vi "20180816 1st Step Analysis.vi"(8 "error in":errorcluster caption="エラー入力", 10 "Set Condition":T8={"+/- Point"=2000, "Cut Region"=500, "BL Selection"=enum."Div Value Mode BL", "STD Selection"=enum."DivSTD Mode STD", "D Th std xn"=1.0, "U Th std xn"=6.0, "MAX D time (ms)"=10.0, "LL BR (n)"=0, "LL BR T length (ms)"=0.0, "LL Retention (ms)"=0.0, "Read Region Point"=10000, "Filter Selection"=enum."Smooth", "STD smooth Point"=10, "MAX E_S time (ms)"=10.0}, 11 "F_name":path=path "D:/MCBJ data/Micro RNA Data/let7f W22/00 Good Signal") -> (0 "error out":errorcluster caption="エラー出力", 2 "Count Graph":cluster{i32[], "Count":dbl[]}[](graph), 3 "Raw data Graph":waveform(dbl)(graph))   [LabVIEW 2018]
uses:
  <vilib>/Analysis/NI_AALBase.lvlib
panel:
  out "stripped path":path
  out "path 2":path
  out "path":path
  out "A New Folder temp":string
  out "Table tmp cluster":T1
  out "Path_Name":T2
  out "tdms tmp path":path
  out "R Pre Burst#":i32
  out "S Table Z":T3
  out "S Anal":cluster{string[], string[], string[]}
  out "Total Burst (s)":dbl
  out "Burst S (n)":i32
  out "AR Table Data":string[](array[string])
  out "AR Table Tag":string[](array[string])
  out "Table Pass refnum":T4
  out "Table Tag C":T5
  out "AA2 info":T6
  out "AR Table Path":path
  out "AA info":T7
  out "before":string
  out "1s datapoint":i32
  in  "Selection":enum16{"10kHz", "100kHz"}(ring)
  out "AC Table Data":string[](array[string])
  out "AC Table Tag":string[](array[string])
  in  "Cut Region":i32=500
  out "info Cluster":T9
  out "R B_SCount [n] in":i32
  out "B Region Time [s] in":dbl
  out "JPEG Path":path
  in  "Region Count":dbl[](array[numeric])
  out "Region BL":dbl[](array[numeric])
  out "TDMS temp refnum":refnum<k34>
  out "S_save C":T10
  out "R Table refnum":refnum<file>
  out "B Table refnum":refnum<file>
  out "S Table refnum":refnum<file>
  out "Burst Pre Count":i32
  out "S Peak Position Final (s)":dbl=1000.0 format="%#_13g"
  out "Signal Pre Count":i32
  out "A TDMS Path":path
  out "B Table Path":path
  out "D con":string
  out "A New folder":string
  out "B Table Tag":string[](array[string])
  out "R Table Tag":string[](array[string])
  out "S Table Tag":string[](array[string])
  out "Burst Array":T11
  out "Burst#Sum":i32
  out "BCC":T12
  in  "MAX E_S time(s)":dbl=0.01 format="%#_13g"
  out "BL and Raw":T13
  in  "LL BR (n)":i32
  in  "LL BR T length (ms)":dbl
  out "Under D array":T14
  out "Peak#":i32
  in  "MAX D time(s)":dbl=0.01 format="%#_13g"
  out "Peak Array":T15
  in  "control":enum32{"Signal", "Region"}(tab)
  out "STD Graph":cluster{i32[], "Count":dbl[]}[](graph)
  out "BL Graph":cluster{i32[], "Count":dbl[]}[](graph)
  out "A Cluster":T16
  out "Signal Freq [/s]":dbl format="%#_4g"
  out "Anal Time":string
  out "Signal TT Graph":T17(graph)
  out "Histogram Graph":T18(graph) caption="ヒストグラムグラフ"
  out "Signal-Time Plot":T19(graph)
  out "Signal-Duration Plot":cluster{i32[], dbl[]}(graph)
  out "Burst Time Profile":cluster{i32[], "SDS":dbl[]}[](graph)
  out "Region Info":T20
  out "AN time":string
  out "Ainfo":string
  out "F ex Info":T21
  out "Ex Time":i32
  out "R Table Path":path
  out "S Table Path":path
  in  "LL Retention (ms)":dbl
  in  "Analysis Table TAB":T22(tab)
  out "S Table":string[][](table)
  out "R Table":string[][](table)
  out "B Table":string[][](table)
  in  "Filter Selection":enum16{"Mean", "Smooth"}(ring)=enum."Smooth"
  in  "+/- Point":i32=2000
  out "Region Raw data":dbl[](array[numeric])
  out "Estimated BL":dbl[](array[numeric])
  out "Substracted Raw data":dbl[](array[numeric])
  in  "BL Selection":T23(ring)=enum."Div Value Mode BL"
  out "Selected Region BL":dbl
  in  "STD Selection":T24(ring)=enum."DivSTD Mode STD"
  out "Selected STD (pA)":dbl
  in  "U Th std xn":dbl=6.0 format="%#_13g"
  in  "D Th std xn":dbl=1.0 format="%#_13g"
  out "Region graph":cluster{"Value":i32[], "UP Thre Func":dbl[]}[](graph)
  out "R Peak location":i32[](array[numeric])
  out "Peak Y":dbl[](array[numeric])
  out "U thred (pA)":dbl
  out "D thred (pA)":dbl
  out "UP Thre Func":dbl[](array[numeric])
  out "Peak G":cluster{"Value":i32[], "Peak Y":dbl[]}
  out "Time for Graph":i32[](array[numeric])
  out "Threshold G":cluster{"Value":i32[], "UP Thre Func":dbl[]}
  out "Raw G":cluster{"Value":i32[], "Peak Y":dbl[]}
  out "BL G":cluster{"Value":i32[], "Value":dbl[]}
  out "Peak Intensity":dbl[](array[numeric])
  out "RS Start":i32[](array[numeric])
  out "RS End":i32[](array[numeric])
  out "Signal Time (ms)":dbl[](array[numeric])
  out "Region Start":i32
  out "TS Peak Time (s)":dbl[](array[numeric])
  out "T Start Time (s)":dbl[](array[numeric])
  out "T END Time (s)":dbl[](array[numeric])
  out "Signal location BL":dbl[](array[numeric])
  out "Filter Select":string
  out "Region BL select":string
  out "R STD select":string
  out "S Table C2":T25={"R BL (pA)"=0.0, "R STD (pA)"=0.0, "U thre (pA)"=0.0, "D thre (pA)"=0.0, "U thre (n)"=0.0, "D thre (n)"=0.0, "STD smoth Point "=10, "MAX Duration time(s)"=0.01} {"MAX Duration time(s)" format="%#_13g"}
  out "S Table C1":T26
  out "S Table C0":T27
  out "Rigon#":i32
  out "BL cluster":T28
  out "HPeak Cluster":T29
  out "STD cluster":T30
  out "R Table C0":T31
  in  "STD smooth Point":i32=10
  out "Signal#Sum":i32
  out "Raw data":dbl[](array[numeric])
  out "Filename":string
  in  "Read Region Point":i32=10000
  out "datapoint":i32
  out "Region STD":dbl[](array[numeric])
  out "Count":dbl[](array[numeric])
  out "STD":dbl[](array[numeric])
  out "BL":dbl[](array[numeric])
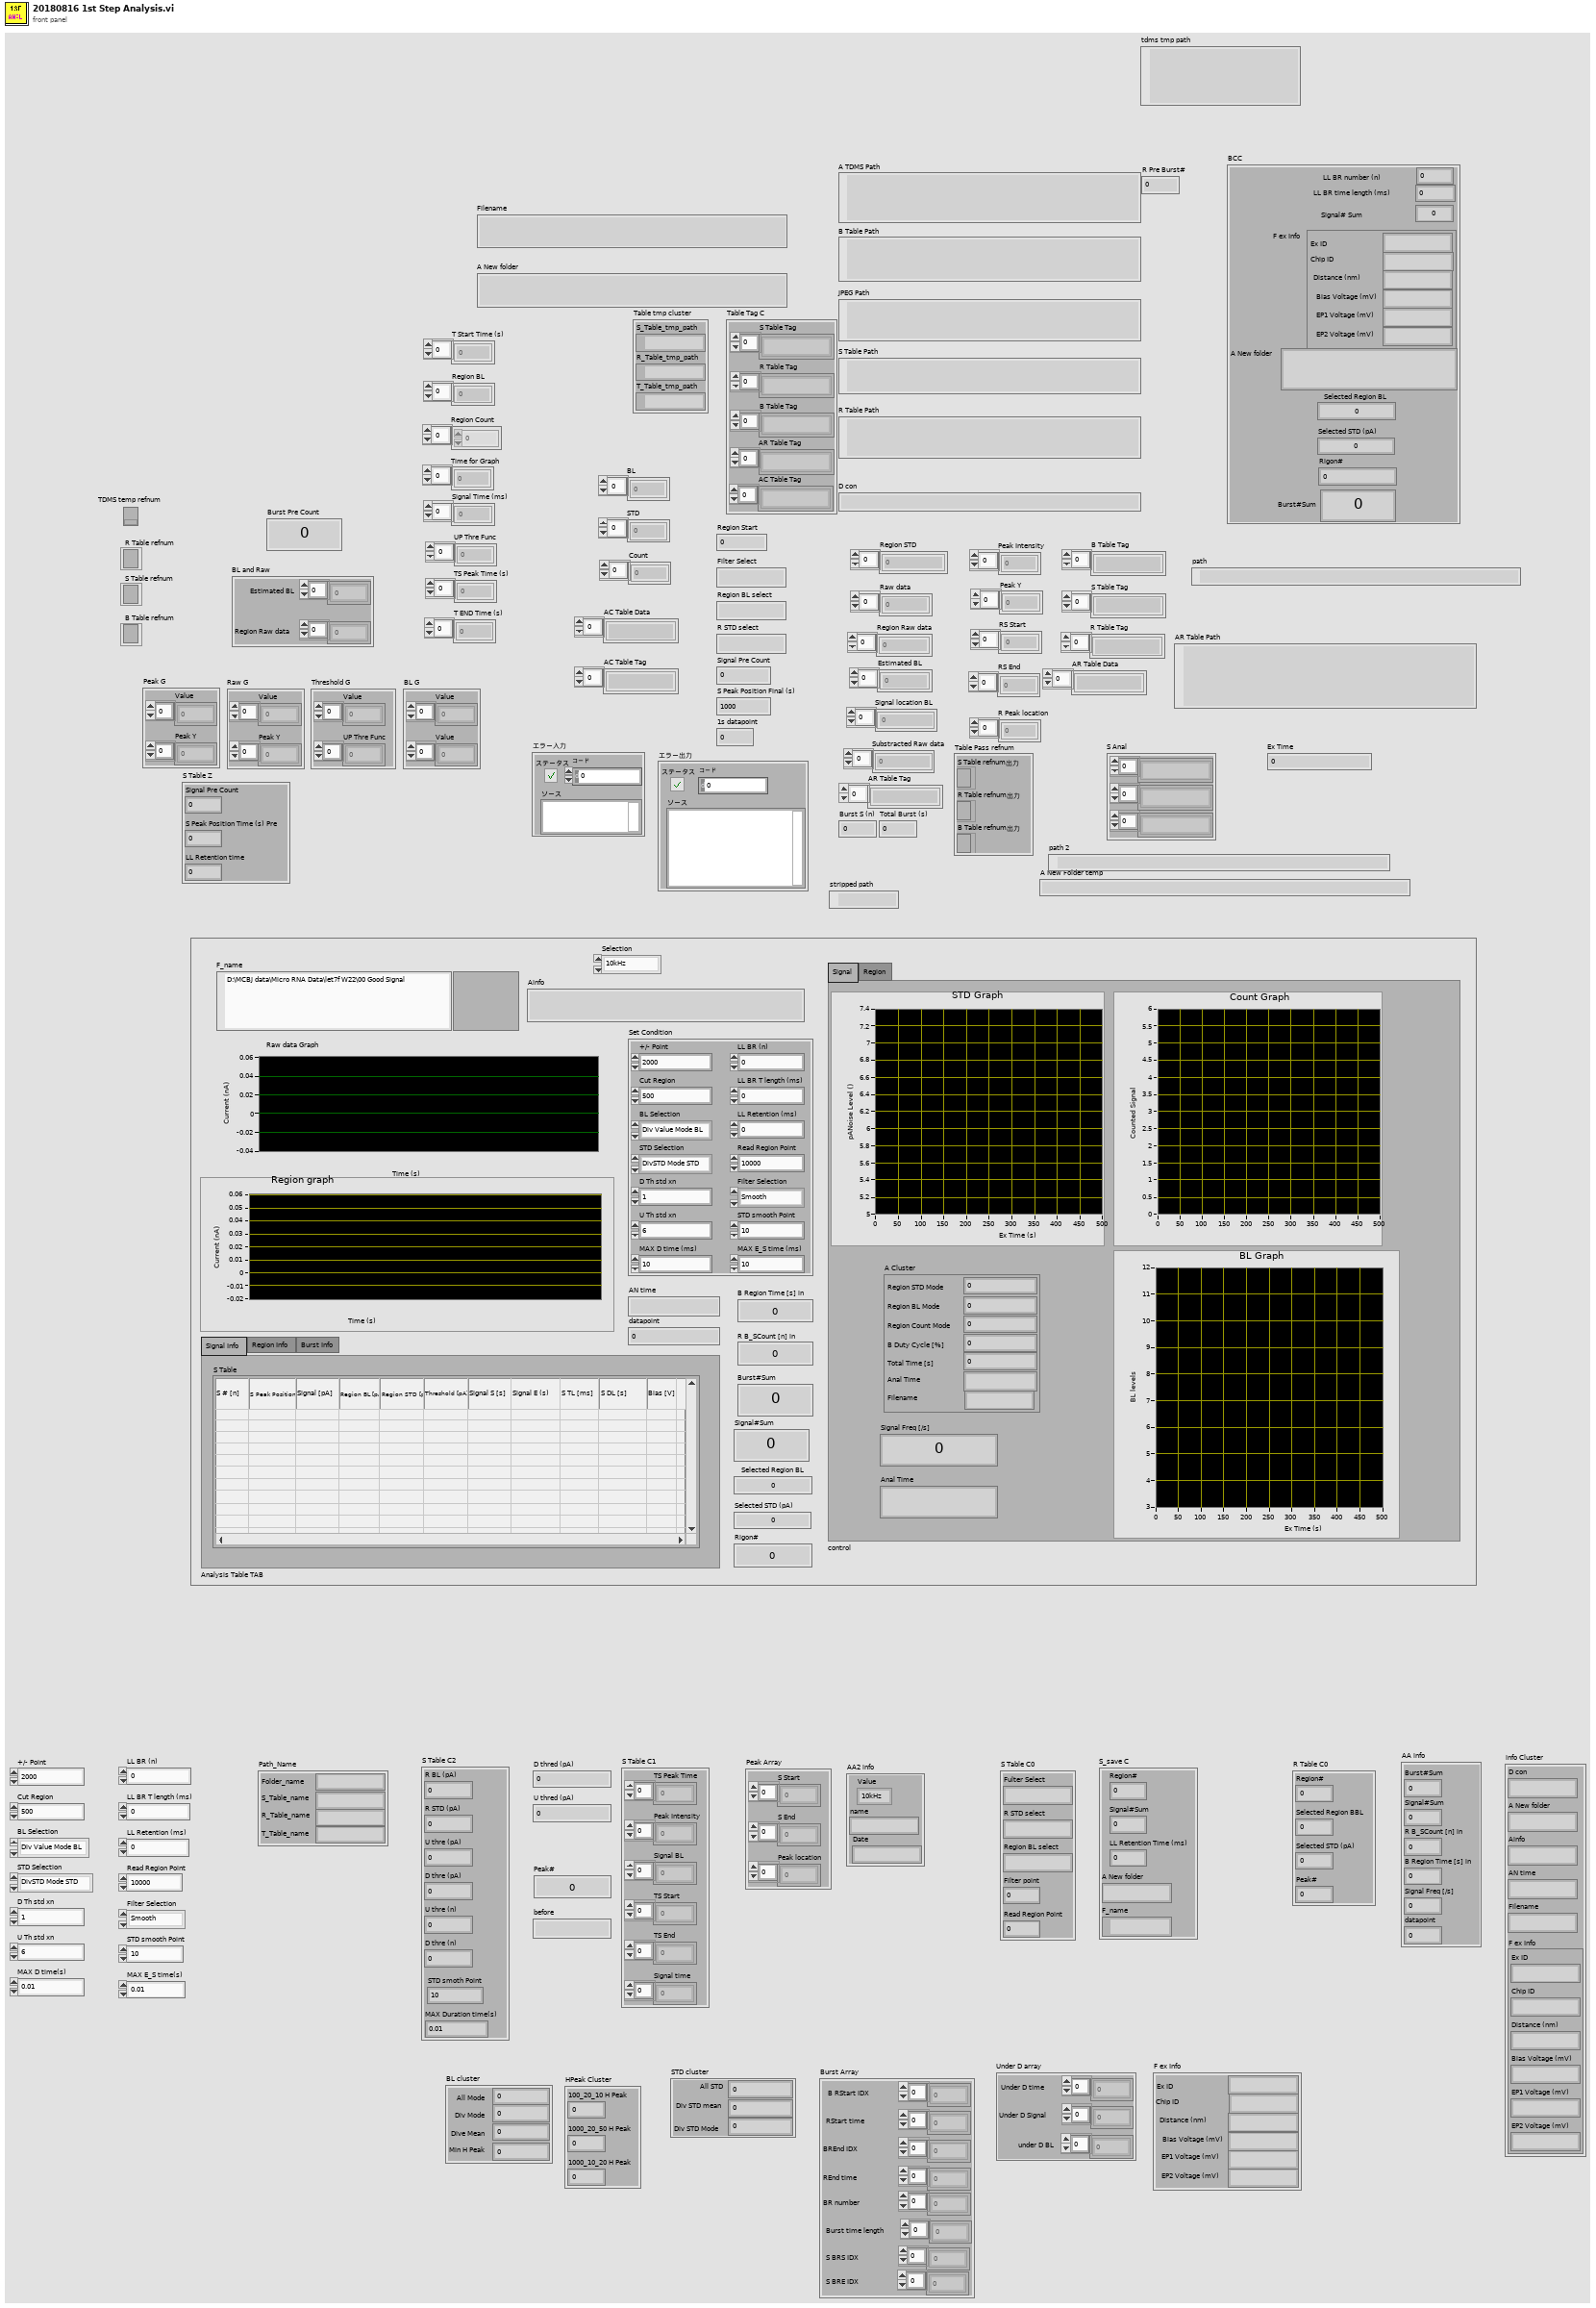
[diagram p1: front panel]
types:
  T1 = cluster{"S_Table_tmp_path":path, "R_Table_tmp_path":path, "T_Table_tmp_path":path}
  T2 = cluster{"Folder_name":string, "S_Table_name":string, "R_Table_name":string, "T_Table_name":string}
  T3 = cluster{"Signal Pre Count":i32, "S Peak Position Time (s) Pre":dbl, "LL Retention time":dbl}
  T4 = cluster{"S Table refnum出力":refnum<file>, "R Table refnum出力":refnum<file>, "B Table refnum出力":refnum<file>}
  T5 = cluster{"S Table Tag":string[], "R Table Tag":string[], "B Table Tag":string[], "AR Table Tag":string[], "AC Table Tag":string[]}
  T6 = cluster{"Value":enum16{"10kHz", "100kHz"}, "name":string, "Date":string}
  T7 = cluster{"Burst#Sum":i32, "Signal#Sum":i32, "R B_SCount [n] in":i32, "B Region Time [s] in":dbl, "Signal Freq [/s]":dbl, "datapoint":i32}
  T8 = cluster{"+/- Point":i32, "Cut Region":i32, "BL Selection":enum16{"All Value Mode BL", "Div Value Mode BL", "Div Mean Mean BL", "Min Peak Value BL"}, "STD Selection":enum16{"All Value STD", "Div STD Mean STD", "DivSTD Mode STD"}, "D Th std xn":dbl, "U Th std xn":dbl, "MAX D time (ms)":dbl, "LL BR (n)":i32, "LL BR T length (ms)":dbl, "LL Retention (ms)":dbl, "Read Region Point":i32, "Filter Selection":enum16{"Mean", "Smooth"}, "STD smooth Point":i32, "MAX E_S time (ms)":dbl}
  T9 = cluster{"D con":string, "A New folder":string, "Ainfo":string, "AN time":string, "Filename":string, "F ex Info":cluster{"Ex ID":string, "Chip ID":string, "Distance (nm)":string, "Bias Voltage (mV)":string, "EP1 Voltage (mV)":string, "EP2 Voltage (mV)":string}}
  T10 = cluster{"Region#":i32, "Signal#Sum":i32, "LL Retention Time (ms)":dbl, "A New folder":string, "F_name":path}
  T11 = cluster{"B RStart IDX":i32[], "RStart time":dbl[], "BREnd IDX":i32[], "REnd time":dbl[], "BR number":dbl[], "Burst time length":dbl[], "S BRS IDX":i32[], "S BRE IDX":i32[]}
  T12 = cluster{"LL BR number (n)":i32, "LL BR time length (ms)":dbl, "Signal# Sum":i32, "F ex Info":cluster{"Ex ID":string, "Chip ID":string, "Distance (nm)":string, "Bias Voltage (mV)":string, "EP1 Voltage (mV)":string, "EP2 Voltage (mV)":string}, "A New folder":string, "Selected STD (pA)":dbl, "Selected Region BL":dbl, "Rigon#":i32, "Burst#Sum":i32}
  T13 = cluster{"Estimated BL":dbl[], "Region Raw data":dbl[]}
  T14 = cluster{"Under D time":dbl[], "Under D Signal":dbl[], "under D BL":dbl[]}
  T15 = cluster{"S Start":i32[], "S End":i32[], "Peak location":i32[]}
  T16 = cluster{"Region STD Mode":dbl, "Region BL Mode":dbl, "Region Count Mode":dbl, "B Duty Cycle [%]":dbl, "Total Time [s]":dbl, "Anal Time":string, "Filename":string}
  T17 = cluster{"TS Start":dbl[], "Peak Intensity":dbl[]}[]
  T18 = cluster{"X Values":dbl[], "Histogram: h(x)":i32[]}
  T19 = cluster{"TS Start":dbl[], "Peak Intensity":dbl[]}
  T20 = cluster{"Signal (n)":i32, "Burst S (n)":i32, "Burst (%)":dbl, "Burst R (n)":dbl, "Mean (pA)":dbl, "STD (pA)":dbl, "SN (%)":dbl, "skewness":dbl, "kurtosis":dbl, "Total Burst (s)":dbl, "B time (%)":dbl}
  T21 = cluster{"Ex ID":string, "Chip ID":string, "Distance (nm)":string, "Bias Voltage (mV)":string, "EP1 Voltage (mV)":string, "EP2 Voltage (mV)":string}
  T22 = enum32{"Signal Info", "Region Info", "Burst Info"}
  T23 = enum16{"All Value Mode BL", "Div Value Mode BL", "Div Mean Mean BL", "Min Peak Value BL"}
  T24 = enum16{"All Value STD", "Div STD Mean STD", "DivSTD Mode STD"}
  T25 = cluster{"R BL (pA)":dbl, "R STD (pA)":dbl, "U thre (pA)":dbl, "D thre (pA)":dbl, "U thre (n)":dbl, "D thre (n)":dbl, "STD smoth Point ":i32, "MAX Duration time(s)":dbl}
  T26 = cluster{"TS Peak Time":dbl[], "Peak Intensity":dbl[], "Signal BL":dbl[], "TS Start":dbl[], "TS End":dbl[], "Signal time":dbl[]}
  T27 = cluster{"Fulter Select":string, "R STD select":string, "Region BL select":string, "Filter point":i32, "Read Region Point":i32}
  T28 = cluster{"All Mode":dbl, "Div Mode":dbl, "Dive Mean":dbl, "Min H Peak":dbl}
  T29 = cluster{"100_20_10 H Peak":i32, "1000_20_50 H Peak":i32, "1000_10_20 H Peak":i32}
  T30 = cluster{"All STD":dbl, "Div STD mean":dbl, "Div STD Mode":dbl}
  T31 = cluster{"Region#":i32, "Selected Region BBL":dbl, "Selected STD (pA)":dbl, "Peak#":i32}
  T32 = enum16{"open", "open or create", "create or replace", "create", "open (read-only)"}
  T33 = cluster{"S Table Pass":path, "R Table Pass":path, "B Table Pass":path, "JPEG Pass":path, "A TDMS Pass":path}
  T34 = cluster{"Value":dbl[], "Value":dbl[], "Value":dbl[], "Value":dbl[], "Value":dbl[], "Value":dbl[]}
  T35 = cluster{"Value":string, "Value":string, "Value":string, "Value":i32, "Value":i32}
  T36 = cluster{"Value":dbl, "Value":dbl, "Value":dbl, "Value":dbl, "Value":dbl, "Value":dbl, "Value":i32, "Value":dbl}
  T37 = cluster{"Value":i32, "Value":dbl, "Value":i32, "Value":cluster{"Ex ID":string, "Chip ID":string, "Distance (nm)":string, "Bias Voltage (mV)":string, "EP1 Voltage (mV)":string, "EP2 Voltage (mV)":string}, "Value":string, "Value":dbl, "Value":dbl, "Value":i32, "Value":i32}
  T38 = cluster{"Value":i32, "Value":i32, "Value":dbl, "Value":string, "Value":path}
  T39 = cluster{"Value":i32, "Value":dbl, "Value":dbl, "Value":i32}
  T40 = cluster{"Value":enum16{"10kHz", "100kHz"}, "name":string, "date/time string":string}
  T41 = cluster{"Value":i32, "Value":i32, "Value":i32, "Value":dbl, "Value":dbl, "Value":i32}
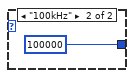
[diagram p2: hidden frame]
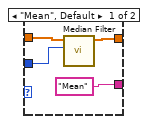
[diagram p3: hidden frame]
diagram:
  w238 = 0.001 ("y")
  w88 = string[][] []
  # "TDMS temp delete"
  # "Temp path formation"
  # "Region Graphe Formation"
  # "check"
  # "check"
  # "S Table Save"
  # "AR Table Formation"
  # "AR Table SAVE"
  # "TXT Table save open"
  # "AC Table save for TDMS"
  # "Original TDMS Data Read"
  # "Tag Formation and TDMS Initialization"
  # "Path Formation"
  # "TXT and TDMS close"
  n1 = Get Date/Time In Seconds() -> (seconds since 1Jan1904=w193:timestamp)
  n2 = call <vilib>:"Clear Errors.vi"("error in (no error)"="error in", "specific error code to clear (0: all)"=6) -> ("error out"=w2:errorcluster)  [unwired: 4 in, 1 out]
  n3 = property on="F_name" class="Path"(error in=w2, "Value"="F_name") -> (error out=w15:errorcluster)  [unwired: 1 in, 1 out]
  n4 = case shown="\"10kHz\", Default" "Selection" {
    tunnel: [10000 ("R B_SCount [n] in") 100000 ("R B_SCount [n] in")] -> w213
    frame "10kHz", Default {
    }
    frame "100kHz" {
    }
  }
  "1s datapoint" <- w213
  n5 = Format Date/Time String(time format string (%c)="%d:%H:%M:%S" ("時間形式文字列（%c）"), seconds (now)=w193) -> (date/time string=w192:string)  [unwired: 1 in]
  n6 = property on="R B_SCount [n] in" class="DigNum (strict)"(error in=w15, "Value"=0 ("R B_SCount [n] in")) -> (error out=w285:errorcluster)  [unwired: 1 in, 1 out]
  n7 = property on="B Region Time [s] in" class="DigNum (strict)"(error in=w285, "Value"=0.0 ("B Region Time [s] in")) -> (error out=w259:errorcluster)  [unwired: 1 in, 1 out]
  n8 = property on="Signal#Sum" class="DigNum (strict)"(error in=w259, "Value"=0 ("Signal#Sum")) -> (error out=w258:errorcluster)  [unwired: 1 in, 1 out]
  n9 = property on="S Peak Position Final (s)" class="DigNum (strict)"(error in=w258, "Value"=0.0 ("S Peak Position Final (s)")) -> (error out=w257:errorcluster)  [unwired: 1 in, 1 out]
  n10 = property on="Signal Pre Count" class="DigNum (strict)"(error in=w257, "Value"=0 ("Signal Pre Count")) -> (error out=w256:errorcluster)  [unwired: 1 in, 1 out]
  n11 = property on="Burst#Sum" class="DigNum (strict)"(error in=w256, "Value"=0 ("Burst#Sum")) -> (error out=w255:errorcluster)  [unwired: 1 in, 1 out]
  n12 = property on="Burst Pre Count" class="DigNum (strict)"(error in=w255, "Value"=0 ("Burst Pre Count")) -> (error out=w87:errorcluster)  [unwired: 1 in, 1 out]
  n13 = property on="R Table" class="Tbl (strict)"(error in=w87, "Value"=w88) -> (error out=w86:errorcluster)  [unwired: 1 in, 1 out]
  n14 = property on="S Table" class="Tbl (strict)"(error in=w86, "Value"=w88) -> (error out=w207:errorcluster)  [unwired: 1 in, 1 out]
  n15 = property on="B Table" class="Tbl (strict)"(error in=w207, "Value"=w88) -> (error out=w206:errorcluster)  [unwired: 1 in, 1 out]
  n16 = property on="BL" class="Arr (strict)"(error in=w206, "Value"=dbl[] [] ("配列")) -> (error out=w205:errorcluster)  [unwired: 1 in, 1 out]
  n17 = property on="STD" class="Arr (strict)"(error in=w205, "Value"=dbl[] [] ("配列")) -> (error out=w204:errorcluster)  [unwired: 1 in, 1 out]
  n18 = property on="Count" class="Arr (strict)"(error in=w204, "Value"=dbl[] [] ("配列")) -> (error out=w203:errorcluster)  [unwired: 1 in, 1 out]
  n19 = property on="Region STD" class="Arr (strict)"(error in=w203, "Value"=dbl[] [] ("配列")) -> (error out=w202:errorcluster)  [unwired: 1 in, 1 out]
  n20 = property on="Region Count" class="Arr (strict)"(error in=w202, "Value"=dbl[] [] ("配列")) -> (error out=w201:errorcluster)  [unwired: 1 in, 1 out]
  n21 = property on="Region BL" class="Arr (strict)"(error in=w201, "Value"=dbl[] [] ("配列")) -> (error out=w190:errorcluster)  [unwired: 1 in, 1 out]
  n22 = property on="before" class="Str"(error in=w190, "Value"="0" ("before")) -> (error out=w189:errorcluster)  [unwired: 1 in, 1 out]
  n23 = Unbundle("Set Condition") -> ("+/- Point"=w254:i32, "Cut Region"=w253:i32, "BL Selection"=w252:T23, "STD Selection"=w251:T24, "D Th std xn"=w250:dbl, "U Th std xn"=w249:dbl, "MAX D time (ms)"=w248:dbl, "LL BR (n)"=w246:i32, "LL BR T length (ms)"=w245:dbl, "LL Retention (ms)"=w244:dbl, "Read Region Point"=w243:i32, "Filter Selection"=w242:enum16{"Mean", "Smooth"}, "STD smooth Point"=w241:i32, "MAX E_S time (ms)"=w240:dbl)
  n24 = property on="before" class="Str"(error in=w189, "Value"=w192) -> (error out=w13:errorcluster)  [unwired: 1 in, 1 out]
  n25 = Multiply(x=w238, y=w240) -> (x*y=w239:dbl)
  n26 = Multiply(x=w248, y=w238) -> (x*y=w247:dbl)
  n27 = property on="F_name" class="Path"(error in=w13) -> (error out=w12:errorcluster, "Value"=w14:path)  [unwired: 1 in, 1 out]
  n28 = property on="+/- Point" class="DigNum (strict)"(error in=w12, "Value"=w254) -> (error out=w237:errorcluster)  [unwired: 1 in, 1 out]
  n29 = property on="Cut Region" class="DigNum (strict)"(error in=w237, "Value"=w253) -> (error out=w236:errorcluster)  [unwired: 1 in, 1 out]
  n30 = property on="BL Selection" class="Enum (strict)"(error in=w236, "Value"=w252) -> (error out=w235:errorcluster)  [unwired: 1 in, 1 out]
  n31 = property on="STD Selection" class="Enum (strict)"(error in=w235, "Value"=w251) -> (error out=w234:errorcluster)  [unwired: 1 in, 1 out]
  n32 = property on="D Th std xn" class="DigNum (strict)"(error in=w234, "Value"=w250) -> (error out=w233:errorcluster)  [unwired: 1 in, 1 out]
  n33 = property on="U Th std xn" class="DigNum (strict)"(error in=w233, "Value"=w249) -> (error out=w232:errorcluster)  [unwired: 1 in, 1 out]
  n34 = property on="MAX D time(s)" class="DigNum (strict)"(error in=w232, "Value"=w247) -> (error out=w231:errorcluster)  [unwired: 1 in, 1 out]
  n35 = property on="LL BR (n)" class="DigNum (strict)"(error in=w231, "Value"=w246) -> (error out=w230:errorcluster)  [unwired: 1 in, 1 out]
  n36 = property on="LL BR T length (ms)" class="DigNum (strict)"(error in=w230, "Value"=w245) -> (error out=w229:errorcluster)  [unwired: 1 in, 1 out]
  n37 = property on="LL Retention (ms)" class="DigNum (strict)"(error in=w229, "Value"=w244) -> (error out=w228:errorcluster)  [unwired: 1 in, 1 out]
  n38 = property on="Read Region Point" class="DigNum (strict)"(error in=w228, "Value"=w243) -> (error out=w227:errorcluster)  [unwired: 1 in, 1 out]
  n39 = property on="Filter Selection" class="Enum (strict)"(error in=w227, "Value"=w242) -> (error out=w226:errorcluster)  [unwired: 1 in, 1 out]
  n40 = property on="STD smooth Point" class="DigNum (strict)"(error in=w226, "Value"=w241) -> (error out=w225:errorcluster)  [unwired: 1 in, 1 out]
  n41 = property on="MAX E_S time(s)" class="DigNum (strict)"(error in=w225, "Value"=w239) -> (error out=w224:errorcluster)  [unwired: 1 in, 1 out]
  n42 = call "ASM A_PATH formation.vi"("error in (no error)"=w224, "F_name"=w14) -> ("error out"=w271:errorcluster, "AR Table Path"=w175:path, "info Cluster"=w280:T9, "SRBJT Path"=w284:T33, "Path_Name"=→"Path_Name":T2)  [unwired: 5 in]
  "info Cluster" <- w280
  n43 = Unbundle(w280) -> ("D con"=w279:string, "A New folder"=w278:string, "Ainfo"=w277:string, "AN time"=w276:string, "Filename"=w275:string, "F ex Info"=w274:T21)
  n44 = Unbundle(w284) -> ("S Table Pass"=w283:path, "R Table Pass"=w282:path, "B Table Pass"=w281:path, "JPEG Pass"=w263:path, "A TDMS Pass"=w262:path)
  n45 = property on="S Table Path" class="Path"(error in=w271, "Value"=w283) -> (error out=w270:errorcluster)  [unwired: 1 in, 1 out]
  n46 = property on="R Table Path" class="Path"(error in=w270, "Value"=w282) -> (error out=w269:errorcluster)  [unwired: 1 in, 1 out]
  n47 = property on="B Table Path" class="Path"(error in=w269, "Value"=w281) -> (error out=w261:errorcluster)  [unwired: 1 in, 1 out]
  n48 = property on="JPEG Path" class="Path"(error in=w261, "Value"=w263) -> (error out=w260:errorcluster)  [unwired: 1 in, 1 out]
  n49 = property on="A TDMS Path" class="Path"(error in=w260, "Value"=w262) -> (error out=w174:errorcluster)  [unwired: 1 in, 1 out]
  n50 = property on="AR Table Path" class="Path"(error in=w174, "Value"=w175) -> (error out=w173:errorcluster)  [unwired: 1 in, 1 out]
  n51 = property on="D con" class="Str"(error in=w173, "Value"=w279) -> (error out=w268:errorcluster)  [unwired: 1 in, 1 out]
  n52 = property on="A New folder" class="Str"(error in=w268, "Value"=w278) -> (error out=w267:errorcluster)  [unwired: 1 in, 1 out]
  n53 = property on="Ainfo" class="Str"(error in=w267, "Value"=w277) -> (error out=w266:errorcluster)  [unwired: 1 in, 1 out]
  n54 = property on="AN time" class="Str"(error in=w266, "Value"=w276) -> (error out=w265:errorcluster)  [unwired: 1 in, 1 out]
  n55 = property on="Filename" class="Str"(error in=w265, "Value"=w275) -> (error out=w264:errorcluster)  [unwired: 1 in, 1 out]
  n56 = property on="F ex Info" class="Clust (strict)"(error in=w264, "Value"=w274) -> (error out=w142:errorcluster)  [unwired: 1 in, 1 out]
  n57 = property on="F_name" class="Path"(error in=w142) -> (error out=w143:errorcluster, "Value"=w273:path)  [unwired: 1 in, 1 out]
  n58 = TDMS Open(8:w143, 10:T32."open or create" ("操作（0:open）"), 11:w273) -> (0:w306:errorcluster, 3:w307:refnum<k34>)  [unwired: 4 in]
  n59 = TDMS Read(0:w307, 11:w306) -> (4:w305:refnum<k34>, 10:w220:waveform(dbl)[], 15:w304:errorcluster)  [unwired: 6 in, 3 out]
  n60 = Array Size(array=w220) -> (size(s)=w222:i32)
  n61 = Decrement(x=w222) -> (x-1=w221:i32)
  n62 = TDMS Close(8:w304, 11:w305) -> (0:w188:errorcluster)  [unwired: 1 out]
  n63 = Index Array(array=w220, index=w221) -> (element=w219:waveform(dbl))
  "Raw data Graph" <- w219
  n64 = Unbundle By Name(w219) -> ("Y"=w137:dbl[])
  n65 = Array Size(array=w137) -> (size(s)=w84:i32)
  n66 = property on="Raw data" class="Arr (strict)"(error in=w188, "Value"=w137) -> (error out=w61:errorcluster)  [unwired: 1 in, 1 out]
  n67 = property on="datapoint" class="DigNum (strict)"(error in=w61, "Value"=w84) -> (error out=w60:errorcluster)  [unwired: 1 in, 1 out]
  n68 = call "temp_test.vi"("error in (no error)"=w60) -> ("error out"=w59:errorcluster, "temp tdms_path B"=w58:path)  [unwired: 6 in, 3 out]
  n69 = property on="tdms tmp path" class="Path"(error in=w59, "Value"=w58) -> (error out=w47:errorcluster)  [unwired: 1 in, 1 out]
  n70 = property on="tdms tmp path" class="Path"(error in=w47) -> (error out=w46:errorcluster, "Value"=w48:path)  [unwired: 1 in, 1 out]
  n71 = property on="Path_Name" class="Clust (strict)"(error in=w46) -> (error out=w45:errorcluster, "Value"=w49:T2)  [unwired: 1 in, 1 out]
  n72 = call "csv temp path.vi"("error in (no error)"=w45, "Path_Name"=w49, "tdms temp path"=w48) -> ("error out"=w44:errorcluster, "A New Folder temp"=w37:string, "Table tmp cluster"=w43:T1)  [unwired: 6 in]
  n73 = property on="Table tmp cluster" class="Clust (strict)"(error in=w44, "Value"=w43) -> (error out=w36:errorcluster)  [unwired: 1 in, 1 out]
  n74 = property on="A New Folder temp" class="Str"(error in=w36, "Value"=w37) -> (error out=w35:errorcluster)  [unwired: 1 in, 1 out]
  n75 = property on="tdms tmp path" class="Path"(error in=w35) -> (error out=w57:errorcluster, "Value"=w56:path)  [unwired: 1 in, 1 out]
  n76 = property on="Raw data" class="Arr (strict)"(error in=w57) -> (error out=w62:errorcluster, "Value"=w144:dbl[])  [unwired: 1 in, 1 out]
  n77 = call "TDMS Initialization and Tag Formation_MS.vi"("error in"=w62, "Raw data"=w144, "A TDMS Pass"=w56) -> ("error out"=w135:errorcluster, "Table Tag C"=w141:T5, "A TDMSファイル出力"=w136:refnum<k34>)  [unwired: 6 in]
  n78 = Unbundle(w141) -> ("S Table Tag"=w140:string[], "R Table Tag"=w63:string[], "B Table Tag"=w139:string[], "AR Table Tag"=w111:string[], "AC Table Tag"=w129:string[])
  n79 = property on="TDMS temp refnum" class="Ref (strict)"(error in=w135, "Value"=w136) -> (error out=w134:errorcluster)  [unwired: 1 in, 1 out]
  n80 = property on="Table Tag C" class="Clust (strict)"(error in=w134, "Value"=w141) -> (error out=w138:errorcluster)  [unwired: 1 in, 1 out]
  n81 = property on="S Table" class="Tbl (strict)"(error in=w138, "Column Headers[]"=w140) -> (error out=w65:errorcluster)  [unwired: 1 in, 1 out]
  n82 = property on="R Table" class="Tbl (strict)"(error in=w65, "Column Headers[]"=w63) -> (error out=w64:errorcluster)  [unwired: 1 in, 1 out]
  n83 = property on="B Table" class="Tbl (strict)"(error in=w64, "Column Headers[]"=w139) -> (error out=w291:errorcluster)  [unwired: 1 in, 1 out]
  n84 = property on="S Table Tag" class="Arr (strict)"(error in=w291, "Value"=w140) -> (error out=w290:errorcluster)  [unwired: 1 in, 1 out]
  n85 = property on="R Table Tag" class="Arr (strict)"(error in=w290, "Value"=w63) -> (error out=w289:errorcluster)  [unwired: 1 in, 1 out]
  n86 = property on="B Table Tag" class="Arr (strict)"(error in=w289, "Value"=w139) -> (error out=w128:errorcluster)  [unwired: 1 in, 1 out]
  n87 = property on="AC Table Tag" class="Arr (strict)"(error in=w128, "Value"=w129) -> (error out=w113:errorcluster)  [unwired: 1 in, 1 out]
  n88 = property on="AR Table Tag" class="Arr (strict)"(error in=w113, "Value"=w111) -> (error out=w112:errorcluster)  [unwired: 1 in, 1 out]
  n89 = property on="TDMS temp refnum" class="Ref (strict)"(error in=w112) -> (error out=w126:errorcluster, "Value"=w131:refnum<k34>)  [unwired: 1 in, 1 out]
  n90 = property on="Set Condition" class="Clust (strict)"(error in=w126) -> (error out=w125:errorcluster, "Value"=w130:T8)  [unwired: 1 in, 1 out]
  n91 = property on="AC Table Tag" class="Arr (strict)"(error in=w125) -> (error out=w124:errorcluster, "Value"=w127:string[])  [unwired: 1 in, 1 out]
  n92 = call "AC Table save for TDMS.vi"("error in"=w124, "AC Table Tag"=w127, "Set Condition"=w130, "TDMSファイル in"=w131) -> ("error out"=w133:errorcluster, "TDMSファイル out"=w132:refnum<k34>)  [unwired: 6 in]
  n93 = property on="TDMS temp refnum" class="Ref (strict)"(error in=w133, "Value"=w132) -> (error out=w121:errorcluster)  [unwired: 1 in, 1 out]
  n94 = property on="Table Tag C" class="Clust (strict)"(error in=w121) -> (error out=w41:errorcluster, "Value"=w123:T5)  [unwired: 1 in, 1 out]
  n95 = property on="Table tmp cluster" class="Clust (strict)"(error in=w41) -> (error out=w40:errorcluster, "Value"=w42:T1)  [unwired: 1 in, 1 out]
  n96 = call "Anal txt open_MS.vi"("Table Tag C"=w123, "error in"=w40, "Table tmp cluster"=w42) -> ("error out"=w122:errorcluster, "Table Pass refnum"=w118:T4)  [unwired: 7 in]
  n97 = Unbundle(w118) -> ("S Table refnum出力"=w294:refnum<file>, "R Table refnum出力"=w216:refnum<file>, "B Table refnum出力"=w215:refnum<file>)
  n98 = property on="S Table refnum" class="Ref (strict)"(error in=w122, "Value"=w294) -> (error out=w218:errorcluster)  [unwired: 1 in, 1 out]
  n99 = property on="R Table refnum" class="Ref (strict)"(error in=w218, "Value"=w216) -> (error out=w217:errorcluster)  [unwired: 1 in, 1 out]
  n100 = property on="B Table refnum" class="Ref (strict)"(error in=w217, "Value"=w215) -> (error out=w117:errorcluster)  [unwired: 1 in, 1 out]
  n101 = property on="Table Pass refnum" class="Clust (strict)"(error in=w117, "Value"=w118) -> (error out=w83:errorcluster)  [unwired: 1 in, 1 out]
  n102 = property on="datapoint" class="DigNum (strict)"(error in=w83) -> (error out=w120:errorcluster, "Value"=w82:i32)  [unwired: 1 in, 1 out]
  n103 = property on="Read Region Point" class="DigNum (strict)"(error in=w120) -> (error out=w119:errorcluster, "Value"=w85:i32)  [unwired: 1 in, 1 out]
  n104 = property on="1s datapoint" class="DigNum (strict)"(error in=w119) -> (error out=w77:errorcluster, "Value"=w209:i32)  [unwired: 1 in, 1 out]
  n105 = Divide(x=w82, y=w85) -> (x/y=w303:dbl)
  n106 = Divide(x=w82, y=w209) -> (x/y=w208:dbl)
  n107 = Round To Nearest(number=w303) -> (nearest integer value=w302:dbl)
  n108 = Reciprocal(x=w209) -> (1/x=w212:dbl)
  n109 = To Long Integer(number=w302) -> (32bit integer=w78:i32)
  n110 = property on="Ex Time" class="DigNum (strict)"(error in=w77, "Value"=w78) -> (error out=w76:errorcluster)  [unwired: 1 in, 1 out]
  n111 = property on="Region graph" class="XYGraph (strict)"(error in=w76, "XScale.Multiplier"=w212) -> (error out=w211:errorcluster)  [unwired: 1 in, 1 out]
  n112 = property on="Raw data Graph" class="WFGraph (strict)"(error in=w211, "XScale.Multiplier"=w212) -> (error out=w210:errorcluster)  [unwired: 1 in, 1 out]
  n113 = property on="Raw data Graph" class="WFGraph (strict)"(error in=w210, "XScale.Maximum"=w208) -> (error out=w81:errorcluster)  [unwired: 1 in, 1 out]
  n114 = property on="Ex Time" class="DigNum (strict)"(error in=w81) -> (error out=w80:errorcluster, "Value"=w79:i32)  [unwired: 1 in, 1 out]
  n115 = for {
    N: w79 -> [_]
    shift-right: [w439] -> w68
    shift-left: w80 -> [w627]
    i -> [w605]
    # "Anal txt save"
    # "Anal Tdms save"
    # "Count for Signal and Burst"
    # "Burst Save and B Table Formation"
    # "Each Signal Save and S Table Preparation"
    # "Burst Save Preparation"
    # "R Table Formation"
    # "Prepartion for R Table Formation"
    # "S Table Formation"
    # "Signal Data C0 For S Table"
    # "Signal Data C2 For S Table"
    # "Peak BL Estimation"
    # "Signal Data C1 For S Table C1"
    # "Region Graph Formation"
    # "Threshold Func for Graph"
    # "Peak location Func for Graph"
    # "Region Analysis: STD Estimation"
    # "Peak Pick-UP Data"
    # "BL substracted Data"
    # "Region Analysis: Baseline Estimation"
    # "Present Read Data Region"
    # "Real-Time Baseline Estimation"
    n116 = property on="Read Region Point" class="DigNum (strict)"(error in=w627) -> (error out=w499:errorcluster, "Value"=w452:i32)  [unwired: 1 in, 1 out]
    n117 = property on="Raw data" class="Arr (strict)"(error in=w499) -> (error out=w446:errorcluster, "Value"=w498:dbl[])  [unwired: 1 in, 1 out]
    n118 = property on="1s datapoint" class="DigNum (strict)"(error in=w446) -> (error out=w445:errorcluster, "Value"=w453:i32)  [unwired: 1 in, 1 out]
    n119 = Divide(x=w453, y=w452) -> (x/y=w450:dbl)
    n120 = Multiply(x=w452, y=w605) -> (x*y=w455:i32)
    "Region Start" <- w455
    n121 = Array Subset(array=w498, index=w455, length=w452) -> (w550:dbl[])
    n122 = Divide(x=w455, y=w452) -> (x/y=w454:dbl)
    n123 = Multiply(x=w450, y=w454) -> (x*y=w451:dbl)
    n124 = property on="Region Raw data" class="Arr (strict)"(error in=w445, "Value"=w550) -> (error out=w549:errorcluster)  [unwired: 1 in, 1 out]
    n125 = property on="Raw data Graph" class="WFGraph (strict)"(error in=w549, "Active Cursor"=u32 0 ("アクティブカーソル"), "Cursor.Cursor X"=w451) -> (error out=w531:errorcluster)  [unwired: 1 in, 1 out]
    n126 = property on="BL Selection" class="Enum (strict)"(error in=w531) -> (error out=w530:errorcluster, "Value"=w532:T23)  [unwired: 1 in, 1 out]
    n127 = property on="Region Raw data" class="Arr (strict)"(error in=w530) -> (error out=w537:errorcluster, "Value"=w548:dbl[])  [unwired: 1 in, 1 out]
    n128 = property on="Cut Region" class="DigNum (strict)"(error in=w537) -> (error out=w521:errorcluster, "Value"=w538:i32)  [unwired: 1 in, 1 out]
    n129 = property on="+/- Point" class="DigNum (strict)"(error in=w521) -> (error out=w520:errorcluster, "Value"=w528:i32)  [unwired: 1 in, 1 out]
    n130 = property on="Filter Selection" class="Enum (strict)"(error in=w520) -> (error out=w518:errorcluster, "Value"=w529:enum16{"Mean", "Smooth"})  [unwired: 1 in, 1 out]
    n131 = call "ASD BL estimation VI.vi"("BL Selection"=w532, "STD Cut"=w538, "Region raw data"=w548) -> ("Selected Region Baseline"=w659:dbl, "Region BL selct"=→"Region BL select":string, "HPeak Cluster"=→"HPeak Cluster":T29, "BL cluster"=→"BL cluster":T28)  [unwired: 5 in]
    n132 = case shown="\"Smooth\"" w529 {
      tunnel: w528 -> [w663 w667]
      tunnel: [w661 w666] -> w544
      tunnel: w548 -> [w662 w665]
      tunnel: ["Mean" "Smooth"] -> w519
      frame "Mean", Default {
        n133 = call <vilib>:"Median Filter.vi"("left rank"=w663, "X"=w662) -> ("Filtered X"=w661:dbl[])  [unwired: 8 in, 1 out]
      }
      frame "Smooth" {
        n134 = call "Smoothing++.vi"("+/- Point"=w667, "Y in"=w665) -> ("Y out"=w666:dbl[])  [unwired: 9 in]
      }
    }
    n135 = To Double Precision Float(number=w659) -> (double precision float=w543:dbl)
    n136 = property on="Estimated BL" class="Arr (strict)"(error in=w518, "Value"=w544) -> (error out=w517:errorcluster)  [unwired: 1 in, 1 out]
    n137 = property on="Filter Select" class="Str"(error in=w517, "Value"=w519) -> (error out=w516:errorcluster)  [unwired: 1 in, 1 out]
    n138 = property on="Selected Region BL" class="DigNum (strict)"(error in=w516, "Value"=w543) -> (error out=w513:errorcluster)  [unwired: 1 in, 1 out]
    n139 = property on="Region Raw data" class="Arr (strict)"(error in=w513) -> (error out=w512:errorcluster, "Value"=w523:dbl[])  [unwired: 1 in, 1 out]
    n140 = property on="Estimated BL" class="Arr (strict)"(error in=w512) -> (error out=w511:errorcluster, "Value"=w522:dbl[])  [unwired: 1 in, 1 out]
    n141 = property on="Cut Region" class="DigNum (strict)"(error in=w511) -> (error out=w510:errorcluster, "Value"=w536:i32)  [unwired: 1 in, 1 out]
    n142 = property on="STD Selection" class="Enum (strict)"(error in=w510) -> (error out=w486:errorcluster, "Value"=w525:T24)  [unwired: 1 in, 1 out]
    n143 = call "ASD Baseline substract VI.vi"("Baseline"=w522, "Region Raw"=w523) -> ("Substracted Raw data"=w488:dbl[])  [unwired: 9 in]
    n144 = call "ASD STD estimation VI.vi"("STD Selection"=w525, "STD Cut"=w536, "BL Substraced raw data"=w488) -> ("Selected STD (pA)"=w514:dbl, "R STD select"=w497:string, "STD cluster"=w489:T30)  [unwired: 6 in]
    n145 = property on="Substracted Raw data" class="Arr (strict)"(error in=w486, "Value"=w488) -> (error out=w485:errorcluster)  [unwired: 1 in, 1 out]
    n146 = property on="STD cluster" class="Clust (strict)"(error in=w485, "Value"=w489) -> (error out=w484:errorcluster)  [unwired: 1 in, 1 out]
    n147 = property on="Selected STD (pA)" class="DigNum (strict)"(error in=w484, "Value"=w514) -> (error out=w496:errorcluster)  [unwired: 1 in, 1 out]
    n148 = property on="R STD select" class="Str"(error in=w496, "Value"=w497) -> (error out=w495:errorcluster)  [unwired: 1 in, 1 out]
    n149 = property on="Region STD" class="Arr (strict)"(error in=w495) -> (error out=w558:errorcluster, "Value"=w598:dbl[])  [unwired: 1 in, 1 out]
    n150 = property on="Region BL" class="Arr (strict)"(error in=w558) -> (error out=w542:errorcluster, "Value"=w559:dbl[])  [unwired: 1 in, 1 out]
    n151 = property on="Selected Region BL" class="DigNum (strict)"(error in=w542) -> (error out=w509:errorcluster, "Value"=w541:dbl)  [unwired: 1 in, 1 out]
    n152 = property on="Selected STD (pA)" class="DigNum (strict)"(error in=w509) -> (error out=w483:errorcluster, "Value"=w515:dbl)  [unwired: 1 in, 1 out]
    n153 = Build Array (concatenate)(w598, w515) -> (w597:dbl[])
    n154 = Build Array (concatenate)(w559, w541) -> (w551:dbl[])
    n155 = property on="Substracted Raw data" class="Arr (strict)"(error in=w483) -> (error out=w482:errorcluster, "Value"=w487:dbl[])  [unwired: 1 in, 1 out]
    n156 = property on="U Th std xn" class="DigNum (strict)"(error in=w482) -> (error out=w506:errorcluster, "Value"=w508:dbl)  [unwired: 1 in, 1 out]
    n157 = property on="D Th std xn" class="DigNum (strict)"(error in=w506) -> (error out=w505:errorcluster, "Value"=w507:dbl)  [unwired: 1 in, 1 out]
    n158 = property on="STD smooth Point" class="DigNum (strict)"(error in=w505) -> (error out=w504:errorcluster, "Value"=w524:i32)  [unwired: 1 in, 1 out]
    n159 = property on="Region STD" class="Arr (strict)"(error in=w504, "Value"=w597) -> (error out=w557:errorcluster)  [unwired: 1 in, 1 out]
    n160 = property on="Region BL" class="Arr (strict)"(error in=w557, "Value"=w551) -> (error out=w556:errorcluster)  [unwired: 1 in, 1 out]
    n161 = property on="Region Start" class="DigNum (strict)"(error in=w556) -> (error out=w547:errorcluster, "Value"=w647:i32)  [unwired: 1 in, 1 out]
    n162 = property on="Estimated BL" class="Arr (strict)"(error in=w547) -> (error out=w546:errorcluster, "Value"=w545:dbl[])  [unwired: 1 in, 1 out]
    n163 = property on="Region Count" class="Arr (strict)"(error in=w546) -> (error out=w469:errorcluster, "Value"=w555:dbl[])  [unwired: 1 in, 1 out]
    n164 = call "ASD STD for Threshold VI.vi"("S Point"=w524, "STD A"=w597) -> ("STD for Thd"=w596:dbl)  [unwired: 9 in]
    n165 = call "ASD Peak-Pick Threshold VI.vi"("D thred std n"=w507, "U thred std n"=w508, "standard deviation (pA)"=w596) -> ("D thred (pA)"=→"D thred (pA)":dbl, "U thred (pA)"=→"U thred (pA)":dbl, "D thred (nA)"=w603:dbl, "U thred (nA)"=w604:dbl)  [unwired: 5 in]
    n166 = call "2Triger Peak detectionM VI.vi"("D Threshold (nA)"=w603, "U Threshold (nA)"=w604, "生データの配列"=w487) -> ("Peak Intensity"=w477:dbl[], "Peak#"=w553:i32, "Peak location"=w586:i32[], "S End"=w587:i32[], "S Start"=w588:i32[])  [unwired: 4 in]
    "R Peak location" <- w586
    "RS Start" <- w588
    "RS End" <- w587
    "Peak#" <- w553
    n167 = Build Array (concatenate)(w555, w553) -> (w554:dbl[])
    n168 = Bundle("S Start"=w588, "S End"=w587, "Peak location"=w586) -> (w527:T15)  [unwired: 1 in]
    n169 = call "ASD Signal SE caluculation VI.vi"("Region Start"=w647, "RS End"=w587, "RS Start"=w588, "R Peak location"=w586) -> ("Signal Time (ms)"=w472:dbl[], "T END Time (s)"=w473:dbl[], "T Start Time (s)"=w479:dbl[], "TS Peak Time (s)"=w481:dbl[])  [unwired: 4 in]
    n170 = call "ASD Signal BL estimation VI.vi"("R Peak location"=w586, "Estimated BL"=w545) -> ("Signal location BL"=w475:dbl[])  [unwired: 9 in]
    n171 = property on="Peak Intensity" class="Arr (strict)"(error in=w469, "Value"=w477) -> (error out=w468:errorcluster)  [unwired: 1 in, 1 out]
    n172 = property on="TS Peak Time (s)" class="Arr (strict)"(error in=w468, "Value"=w481) -> (error out=w467:errorcluster)  [unwired: 1 in, 1 out]
    n173 = property on="T Start Time (s)" class="Arr (strict)"(error in=w467, "Value"=w479) -> (error out=w466:errorcluster)  [unwired: 1 in, 1 out]
    n174 = property on="T END Time (s)" class="Arr (strict)"(error in=w466, "Value"=w473) -> (error out=w465:errorcluster)  [unwired: 1 in, 1 out]
    n175 = property on="Signal Time (ms)" class="Arr (strict)"(error in=w465, "Value"=w472) -> (error out=w464:errorcluster)  [unwired: 1 in, 1 out]
    n176 = property on="Region Count" class="Arr (strict)"(error in=w464, "Value"=w554) -> (error out=w463:errorcluster)  [unwired: 1 in, 1 out]
    n177 = property on="Peak Array" class="Clust (strict)"(error in=w463, "Value"=w527) -> (error out=w462:errorcluster)  [unwired: 1 in, 1 out]
    n178 = property on="Signal location BL" class="Arr (strict)"(error in=w462, "Value"=w475) -> (error out=w461:errorcluster)  [unwired: 1 in, 1 out]
    n179 = property on="Region Raw data" class="Arr (strict)"(error in=w461) -> (error out=w326:errorcluster, "Value"=w539:dbl[])  [unwired: 1 in, 1 out]
    n180 = property on="Estimated BL" class="Arr (strict)"(error in=w326) -> (error out=w626:errorcluster, "Value"=w656:dbl[])  [unwired: 1 in, 1 out]
    n181 = property on="U thred (pA)" class="DigNum (strict)"(error in=w626) -> (error out=w625:errorcluster, "Value"=w655:dbl)  [unwired: 1 in, 1 out]
    n182 = property on="D thred (pA)" class="DigNum (strict)"(error in=w625) -> (error out=w325:errorcluster, "Value"=w654:dbl)  [unwired: 1 in, 1 out]
    n183 = property on="Time for Graph" class="Arr (strict)"(error in=w325) -> (error out=w624:errorcluster, "Value"=w650:i32[])  [unwired: 1 in, 1 out]
    n184 = property on="Estimated BL" class="Arr (strict)"(error in=w624) -> (error out=w324:errorcluster, "Value"=w649:dbl[])  [unwired: 1 in, 1 out]
    n185 = call "ASD Peak location for Graph VI.vi"("Peak Locations"=w586, "Region Raw data"=w539) -> ("Peak Y"=w653:dbl[])  [unwired: 9 in]
    "Peak Y" <- w653
    n186 = call "ASD Time point for Graph VI.vi"("Region Raw data"=w539) -> ("Time for Graph"=w651:i32[])  [unwired: 10 in]
    "Time for Graph" <- w651
    n187 = call "ASD Threshold Function VI.vi"("D thred (pA)"=w654, "U thred (pA)"=w655, "Estimated BL"=w656) -> ("UP Thre Func"=w652:dbl[])  [unwired: 7 in, 1 out]
    "UP Thre Func" <- w652
    n188 = Bundle("Time for Graph"=w651, "Value"=w539) -> (w601:cluster{"Time for Graph":i32[], "Value":dbl[]})  [unwired: 1 in]
    "Raw G" <- w601
    n189 = Bundle("Peak location"=w586, "Peak Y"=w653) -> (w600:cluster{"Peak location":i32[], "Peak Y":dbl[]})  [unwired: 1 in]
    "Peak G" <- w600
    n190 = Bundle("Value"=w650, "UP Thre Func"=w652) -> (w599:cluster{"Value":i32[], "UP Thre Func":dbl[]})  [unwired: 1 in]
    "Threshold G" <- w599
    n191 = Bundle("Value"=w650, "Value"=w649) -> (w602:cluster{"Value":i32[], "Value":dbl[]})  [unwired: 1 in]
    "BL G" <- w602
    n192 = Build Array(w602, w601, w600, w599) -> (→"Region graph":cluster{"Value":i32[], "UP Thre Func":dbl[]}[])
    n193 = property on="TS Peak Time (s)" class="Arr (strict)"(error in=w324) -> (error out=w323:errorcluster, "Value"=w480:dbl[])  [unwired: 1 in, 1 out]
    n194 = property on="Peak Intensity" class="Arr (strict)"(error in=w323) -> (error out=w460:errorcluster, "Value"=w476:dbl[])  [unwired: 1 in, 1 out]
    n195 = property on="Signal location BL" class="Arr (strict)"(error in=w460) -> (error out=w459:errorcluster, "Value"=w474:dbl[])  [unwired: 1 in, 1 out]
    n196 = property on="T Start Time (s)" class="Arr (strict)"(error in=w459) -> (error out=w322:errorcluster, "Value"=w478:dbl[])  [unwired: 1 in, 1 out]
    n197 = property on="T END Time (s)" class="Arr (strict)"(error in=w322) -> (error out=w458:errorcluster, "Value"=w470:dbl[])  [unwired: 1 in, 1 out]
    n198 = property on="Signal Time (ms)" class="Arr (strict)"(error in=w458) -> (error out=w457:errorcluster, "Value"=w471:dbl[])  [unwired: 1 in, 1 out]
    n199 = Bundle("Value"=w480, "Value"=w476, "Value"=w474, "Value"=w478, "Value"=w470, "Value"=w471) -> (w492:T34)  [unwired: 1 in]
    n200 = property on="S Table C1" class="Clust (strict)"(error in=w457, "Value"=w492) -> (error out=w321:errorcluster)  [unwired: 1 in, 1 out]
    n201 = property on="Filter Select" class="Str"(error in=w321) -> (error out=w623:errorcluster, "Value"=w638:string)  [unwired: 1 in, 1 out]
    n202 = property on="R STD select" class="Str"(error in=w623) -> (error out=w622:errorcluster, "Value"=w637:string)  [unwired: 1 in, 1 out]
    n203 = property on="Region BL select" class="Str"(error in=w622) -> (error out=w621:errorcluster, "Value"=w636:string)  [unwired: 1 in, 1 out]
    n204 = property on="+/- Point" class="DigNum (strict)"(error in=w621) -> (error out=w620:errorcluster, "Value"=w635:i32)  [unwired: 1 in, 1 out]
    n205 = property on="Read Region Point" class="DigNum (strict)"(error in=w620) -> (error out=w494:errorcluster, "Value"=w634:i32)  [unwired: 1 in, 1 out]
    n206 = Bundle("Value"=w638, "Value"=w637, "Value"=w636, "Value"=w635, "Value"=w634) -> (→"S Table C0":T35)  [unwired: 1 in]
    n207 = property on="S Table C1" class="Clust (strict)"(error in=w494) -> (error out=w493:errorcluster, "Value"=w491:T26)  [unwired: 1 in, 1 out]
    n208 = property on="MAX E_S time(s)" class="DigNum (strict)"(error in=w493) -> (error out=w501:errorcluster, "Value"=w503:dbl)  [unwired: 1 in, 1 out]
    n209 = property on="MAX D time(s)" class="DigNum (strict)"(error in=w501) -> (error out=w500:errorcluster, "Value"=w502:dbl)  [unwired: 1 in, 1 out]
    n210 = property on="Selected Region BL" class="DigNum (strict)"(error in=w500) -> (error out=w619:errorcluster, "Value"=w645:dbl)  [unwired: 1 in, 1 out]
    n211 = property on="Selected STD (pA)" class="DigNum (strict)"(error in=w619) -> (error out=w618:errorcluster, "Value"=w644:dbl)  [unwired: 1 in, 1 out]
    n212 = property on="U thred (pA)" class="DigNum (strict)"(error in=w618) -> (error out=w617:errorcluster, "Value"=w643:dbl)  [unwired: 1 in, 1 out]
    n213 = property on="D thred (pA)" class="DigNum (strict)"(error in=w617) -> (error out=w616:errorcluster, "Value"=w642:dbl)  [unwired: 1 in, 1 out]
    n214 = property on="U Th std xn" class="DigNum (strict)"(error in=w616) -> (error out=w615:errorcluster, "Value"=w641:dbl)  [unwired: 1 in, 1 out]
    n215 = property on="D Th std xn" class="DigNum (strict)"(error in=w615) -> (error out=w535:errorcluster, "Value"=w640:dbl)  [unwired: 1 in, 1 out]
    n216 = property on="STD smooth Point" class="DigNum (strict)"(error in=w535) -> (error out=w534:errorcluster, "Value"=w533:i32)  [unwired: 1 in, 1 out]
    n217 = property on="MAX D time(s)" class="DigNum (strict)"(error in=w534) -> (error out=w435:errorcluster, "Value"=w580:dbl)  [unwired: 1 in, 1 out]
    n218 = Bundle("Value"=w645, "Value"=w644, "Value"=w643, "Value"=w642, "Value"=w641, "Value"=w640, "Value"=w533, "Value"=w580) -> (→"S Table C2":T36)  [unwired: 1 in]
    n219 = call "region analysis.vi"("MAX Duration time(s)"=w502, "MAX E and S time(s)"=w503, "S Table C1"=w491) -> ("All Signal Intensity Histogram"=→"Histogram Graph":T18, "D-I Graph"=→"Signal-Time Plot":T19, "Duration Graph"=→"Signal-Duration Plot":cluster{i32[], dbl[]}, "STD Graph"=→"Signal TT Graph":T17, "Burst Array"=w382:T11, "Burst Time Profile"=→"Burst Time Profile":cluster{i32[], "SDS":dbl[]}[], "Under D array"=w383:T14, "Region Info"=w438:T20)  [unwired: 1 in]
    n220 = Unbundle(w438) -> ("Burst S (n)"=w437:i32, "Total Burst (s)"=w436:dbl)  [unwired: 9 out]
    n221 = property on="Region Info" class="Clust (strict)"(error in=w435, "Value"=w438) -> (error out=w434:errorcluster)  [unwired: 1 in, 1 out]
    n222 = property on="Burst S (n)" class="DigNum (strict)"(error in=w434, "Value"=w437) -> (error out=w433:errorcluster)  [unwired: 1 in, 1 out]
    n223 = property on="Total Burst (s)" class="DigNum (strict)"(error in=w433, "Value"=w436) -> (error out=w381:errorcluster)  [unwired: 1 in, 1 out]
    n224 = property on="Under D array" class="Clust (strict)"(error in=w381, "Value"=w383) -> (error out=w380:errorcluster)  [unwired: 1 in, 1 out]
    n225 = property on="Burst Array" class="Clust (strict)"(error in=w380, "Value"=w382) -> (error out=w379:errorcluster)  [unwired: 1 in, 1 out]
    n226 = property on="LL BR (n)" class="DigNum (strict)"(error in=w379) -> (error out=w581:errorcluster, "Value"=w582:i32)  [unwired: 1 in, 1 out]
    n227 = property on="LL BR T length (ms)" class="DigNum (strict)"(error in=w581) -> (error out=w363:errorcluster, "Value"=w583:dbl)  [unwired: 1 in, 1 out]
    n228 = property on="Signal#Sum" class="DigNum (strict)"(error in=w363) -> (error out=w575:errorcluster, "Value"=w577:i32)  [unwired: 1 in, 1 out]
    n229 = property on="F ex Info" class="Clust (strict)"(error in=w575) -> (error out=w318:errorcluster, "Value"=w576:T21)  [unwired: 1 in, 1 out]
    n230 = property on="A New Folder temp" class="Str"(error in=w318) -> (error out=w317:errorcluster, "Value"=w316:string)  [unwired: 1 in, 1 out]
    n231 = property on="Selected STD (pA)" class="DigNum (strict)"(error in=w317) -> (error out=w574:errorcluster, "Value"=w573:dbl)  [unwired: 1 in, 1 out]
    n232 = property on="Selected Region BL" class="DigNum (strict)"(error in=w574) -> (error out=w570:errorcluster, "Value"=w572:dbl)  [unwired: 1 in, 1 out]
    n233 = property on="Rigon#" class="DigNum (strict)"(error in=w570) -> (error out=w362:errorcluster, "Value"=w571:i32)  [unwired: 1 in, 1 out]
    n234 = property on="Burst#Sum" class="DigNum (strict)"(error in=w362) -> (error out=w361:errorcluster, "Value"=w561:i32)  [unwired: 1 in, 1 out]
    n235 = property on="Estimated BL" class="Arr (strict)"(error in=w361) -> (error out=w360:errorcluster, "Value"=w579:dbl[])  [unwired: 1 in, 1 out]
    n236 = property on="Region Raw data" class="Arr (strict)"(error in=w360) -> (error out=w359:errorcluster, "Value"=w578:dbl[])  [unwired: 1 in, 1 out]
    n237 = Bundle("Value"=w579, "Value"=w578) -> (w365:cluster{"Value":dbl[], "Value":dbl[]})  [unwired: 1 in]
    n238 = Bundle("Value"=w582, "Value"=w583, "Value"=w577, "Value"=w576, "Value"=w316, "Value"=w573, "Value"=w572, "Value"=w571, "Value"=w561) -> (w367:T37)  [unwired: 1 in]
    n239 = property on="BCC" class="Clust (strict)"(error in=w359, "Value"=w367) -> (error out=w358:errorcluster)  [unwired: 1 in, 1 out]
    n240 = property on="BL and Raw" class="Clust (strict)"(error in=w358, "Value"=w365) -> (error out=w357:errorcluster)  [unwired: 1 in, 1 out]
    n241 = property on="BL and Raw" class="Clust (strict)"(error in=w357) -> (error out=w356:errorcluster, "Value"=w364:T13)  [unwired: 1 in, 1 out]
    n242 = property on="BCC" class="Clust (strict)"(error in=w356) -> (error out=w355:errorcluster, "Value"=w366:T12)  [unwired: 1 in, 1 out]
    n243 = property on="F_name" class="Path"(error in=w355) -> (error out=w354:errorcluster, "Value"=w371:path)  [unwired: 1 in, 1 out]
    n244 = property on="Burst Array" class="Clust (strict)"(error in=w354) -> (error out=w353:errorcluster, "Value"=w370:T11)  [unwired: 1 in, 1 out]
    n245 = property on="Under D array" class="Clust (strict)"(error in=w353) -> (error out=w311:errorcluster, "Value"=w369:T14)  [unwired: 1 in, 1 out]
    n246 = call "S_ASD Each Burst SAVE Modified_MS VI.vi"("BL and Raw"=w364, "BCC"=w366, "error in"=w311, "Under D array"=w369, "Burst Array"=w370, "Filename"=w371) -> ("error out"=w310:errorcluster, "R Burst#"=w378:i32, "B Table"=w368:string[][])  [unwired: 3 in]
    n247 = property on="B Table" class="Tbl (strict)"(error in=w310, "Value"=w368) -> (error out=w352:errorcluster)  [unwired: 1 in, 1 out]
    n248 = property on="R Pre Burst#" class="DigNum (strict)"(error in=w352, "Value"=w378) -> (error out=w351:errorcluster)  [unwired: 1 in, 1 out]
    n249 = property on="Peak Array" class="Clust (strict)"(error in=w351) -> (error out=w526:errorcluster, "Value"=w442:T15)  [unwired: 1 in, 1 out]
    n250 = property on="Region Raw data" class="Arr (strict)"(error in=w526) -> (error out=w594:errorcluster, "Value"=w440:dbl[])  [unwired: 1 in, 1 out]
    n251 = property on="Rigon#" class="DigNum (strict)"(error in=w594) -> (error out=w595:errorcluster, "Value"=w562:i32)  [unwired: 1 in, 1 out]
    n252 = property on="LL Retention (ms)" class="DigNum (strict)"(error in=w595) -> (error out=w569:errorcluster, "Value"=w564:dbl)  [unwired: 1 in, 1 out]
    n253 = property on="F_name" class="Path"(error in=w569) -> (error out=w315:errorcluster, "Value"=w563:path)  [unwired: 1 in, 1 out]
    n254 = property on="A New Folder temp" class="Str"(error in=w315) -> (error out=w314:errorcluster, "Value"=w313:string)  [unwired: 1 in, 1 out]
    n255 = property on="Signal#Sum" class="DigNum (strict)"(error in=w314) -> (error out=w490:errorcluster, "Value"=w565:i32)  [unwired: 1 in, 1 out]
    n256 = property on="S Table C1" class="Clust (strict)"(error in=w490) -> (error out=w444:errorcluster, "Value"=w443:T26)  [unwired: 1 in, 1 out]
    n257 = Bundle("Value"=w562, "Value"=w565, "Value"=w564, "Value"=w313, "Value"=w563) -> (w441:T38)  [unwired: 1 in]
    "S_save C" <- w441
    n258 = call "S_ASD Each Signal SAVE_MS VI.vi"("Peak Array"=w442, "error in"=w444, "S Table C1"=w443, "Region raw data"=w440, "S_save C"=w441) -> ("error out"=w417:errorcluster, "S Anal"=w416:cluster{string[], string[], string[]})  [unwired: 4 in, 1 out]
    n259 = property on="S Anal" class="Clust (strict)"(error in=w417, "Value"=w416) -> (error out=w415:errorcluster)  [unwired: 1 in, 1 out]
    n260 = property on="S Anal" class="Clust (strict)"(error in=w415) -> (error out=w414:errorcluster, "Value"=w400:cluster{string[], string[], string[]})  [unwired: 1 in, 1 out]
    n261 = property on="S Table C0" class="Clust (strict)"(error in=w414) -> (error out=w614:errorcluster, "Value"=w418:T27)  [unwired: 1 in, 1 out]
    n262 = property on="S Table C1" class="Clust (strict)"(error in=w614) -> (error out=w613:errorcluster, "Value"=w404:T26)  [unwired: 1 in, 1 out]
    n263 = property on="S Table C2" class="Clust (strict)"(error in=w613) -> (error out=w593:errorcluster, "Value"=w403:T25)  [unwired: 1 in, 1 out]
    n264 = property on="F ex Info" class="Clust (strict)"(error in=w593) -> (error out=w396:errorcluster, "Value"=w401:T21)  [unwired: 1 in, 1 out]
    n265 = property on="Signal#Sum" class="DigNum (strict)"(error in=w396) -> (error out=w395:errorcluster, "Value"=w552:i32)  [unwired: 1 in, 1 out]
    n266 = property on="S Peak Position Final (s)" class="DigNum (strict)"(error in=w395) -> (error out=w394:errorcluster, "Value"=w566:dbl)  [unwired: 1 in, 1 out]
    n267 = property on="LL Retention (ms)" class="DigNum (strict)"(error in=w394) -> (error out=w393:errorcluster, "Value"=w567:dbl)  [unwired: 1 in, 1 out]
    n268 = Bundle("Value"=w552, "Value"=w566, "Value"=w567) -> (w413:cluster{"Value":i32, "Value":dbl, "Value":dbl})  [unwired: 1 in]
    "S Table Z" <- w413
    n269 = call "ASDE Signal Data Table For New_MS.vi"("S Anal"=w400, "F ex Info"=w401, "S Table Z"=w413, "error in"=w393, "S Table C2"=w403, "S Table C1"=w404, "S Table C0"=w418) -> ("error out"=w412:errorcluster, "S Peak Position Final (s)"=w411:dbl, "Signal R count (n)"=w408:i32, "S Table Present Sum"=w402:string[][])  [unwired: 1 in]
    n270 = property on="S Table" class="Tbl (strict)"(error in=w412, "Value"=w402) -> (error out=w399:errorcluster)  [unwired: 1 in, 1 out]
    n271 = property on="Signal Pre Count" class="DigNum (strict)"(error in=w399, "Value"=w408) -> (error out=w398:errorcluster)  [unwired: 1 in, 1 out]
    n272 = property on="S Peak Position Final (s)" class="DigNum (strict)"(error in=w398, "Value"=w411) -> (error out=w397:errorcluster)  [unwired: 1 in, 1 out]
    n273 = property on="Rigon#" class="DigNum (strict)"(error in=w397) -> (error out=w612:errorcluster, "Value"=w631:i32)  [unwired: 1 in, 1 out]
    n274 = property on="Selected Region BL" class="DigNum (strict)"(error in=w612) -> (error out=w611:errorcluster, "Value"=w630:dbl)  [unwired: 1 in, 1 out]
    n275 = property on="Selected STD (pA)" class="DigNum (strict)"(error in=w611) -> (error out=w610:errorcluster, "Value"=w629:dbl)  [unwired: 1 in, 1 out]
    n276 = property on="Peak#" class="DigNum (strict)"(error in=w610) -> (error out=w319:errorcluster, "Value"=w628:i32)  [unwired: 1 in, 1 out]
    n277 = Bundle("Value"=w631, "Value"=w630, "Value"=w629, "Value"=w628) -> (→"R Table C0":T39)  [unwired: 1 in]
    n278 = property on="F ex Info" class="Clust (strict)"(error in=w319) -> (error out=w421:errorcluster, "Value"=w426:T21)  [unwired: 1 in, 1 out]
    n279 = property on="R Table C0" class="Clust (strict)"(error in=w421) -> (error out=w609:errorcluster, "Value"=w312:T31)  [unwired: 1 in, 1 out]
    n280 = property on="BL cluster" class="Clust (strict)"(error in=w609) -> (error out=w608:errorcluster, "Value"=w425:T28)  [unwired: 1 in, 1 out]
    n281 = property on="STD cluster" class="Clust (strict)"(error in=w608) -> (error out=w607:errorcluster, "Value"=w424:T30)  [unwired: 1 in, 1 out]
    n282 = property on="HPeak Cluster" class="Clust (strict)"(error in=w607) -> (error out=w584:errorcluster, "Value"=w423:T29)  [unwired: 1 in, 1 out]
    n283 = property on="Region Info" class="Clust (strict)"(error in=w584) -> (error out=w419:errorcluster, "Value"=w422:T20)  [unwired: 1 in, 1 out]
    n284 = call "R Table data formation.vi"("Region Info"=w422, "F ex Info"=w426, "HPeak Cluster"=w423, "STD cluster"=w424, "BL cluster"=w425, "R Table C0"=w312) -> ("appended array"=w420:string[][])  [unwired: 5 in]
    n285 = property on="R Table" class="Tbl (strict)"(error in=w419, "Value"=w420) -> (error out=w392:errorcluster)  [unwired: 1 in, 1 out]
    n286 = property on="Total Burst (s)" class="DigNum (strict)"(error in=w392) -> (error out=w391:errorcluster, "Value"=w432:dbl)  [unwired: 1 in, 1 out]
    n287 = property on="B Region Time [s] in" class="DigNum (strict)"(error in=w391) -> (error out=w390:errorcluster, "Value"=w431:dbl)  [unwired: 1 in, 1 out]
    n288 = property on="Burst S (n)" class="DigNum (strict)"(error in=w390) -> (error out=w389:errorcluster, "Value"=w429:i32)  [unwired: 1 in, 1 out]
    n289 = property on="R B_SCount [n] in" class="DigNum (strict)"(error in=w389) -> (error out=w388:errorcluster, "Value"=w428:i32)  [unwired: 1 in, 1 out]
    n290 = property on="Signal#Sum" class="DigNum (strict)"(error in=w388) -> (error out=w387:errorcluster, "Value"=w410:i32)  [unwired: 1 in, 1 out]
    n291 = property on="Signal Pre Count" class="DigNum (strict)"(error in=w387) -> (error out=w386:errorcluster, "Value"=w407:i32)  [unwired: 1 in, 1 out]
    n292 = property on="Rigon#" class="DigNum (strict)"(error in=w386) -> (error out=w375:errorcluster, "Value"=w406:i32)  [unwired: 1 in, 1 out]
    n293 = property on="Burst#Sum" class="DigNum (strict)"(error in=w375) -> (error out=w374:errorcluster, "Value"=w377:i32)  [unwired: 1 in, 1 out]
    n294 = property on="R Pre Burst#" class="DigNum (strict)"(error in=w374) -> (error out=w373:errorcluster, "Value"=w376:i32)  [unwired: 1 in, 1 out]
    n295 = Add(x=w410, y=w407) -> (x+y=w409:i32)
    n296 = Add(x=w432, y=w431) -> (x+y=w430:dbl)
    n297 = Add(x=w377, y=w376) -> (x+y=w568:i32)
    n298 = Add(x=w429, y=w428) -> (x+y=w427:i32)
    n299 = Divide(x=w409, y=w406) -> (x/y=w405:dbl)
    n300 = property on="B Region Time [s] in" class="DigNum (strict)"(error in=w373, "Value"=w430) -> (error out=w540:errorcluster)  [unwired: 1 in, 1 out]
    n301 = property on="R B_SCount [n] in" class="DigNum (strict)"(error in=w540, "Value"=w427) -> (error out=w385:errorcluster)  [unwired: 1 in, 1 out]
    n302 = property on="Signal#Sum" class="DigNum (strict)"(error in=w385, "Value"=w409) -> (error out=w384:errorcluster)  [unwired: 1 in, 1 out]
    n303 = property on="Signal Freq [/s]" class="DigNum (strict)"(error in=w384, "Value"=w405) -> (error out=w372:errorcluster)  [unwired: 1 in, 1 out]
    n304 = property on="Burst#Sum" class="DigNum (strict)"(error in=w372, "Value"=w568) -> (error out=w327:errorcluster)  [unwired: 1 in, 1 out]
    n305 = property on="TDMS temp refnum" class="Ref (strict)"(error in=w327) -> (error out=w344:errorcluster, "Value"=w349:refnum<k34>)  [unwired: 1 in, 1 out]
    n306 = property on="Table Tag C" class="Clust (strict)"(error in=w344) -> (error out=w343:errorcluster, "Value"=w348:T5)  [unwired: 1 in, 1 out]
    n307 = property on="S Table" class="Tbl (strict)"(error in=w343) -> (error out=w342:errorcluster, "Value"=w347:string[][])  [unwired: 1 in, 1 out]
    n308 = property on="R Table" class="Tbl (strict)"(error in=w342) -> (error out=w341:errorcluster, "Value"=w346:string[][])  [unwired: 1 in, 1 out]
    n309 = property on="B Table" class="Tbl (strict)"(error in=w341) -> (error out=w340:errorcluster, "Value"=w345:string[][])  [unwired: 1 in, 1 out]
    n310 = call "Anal tdms each save.vi"("B Table"=w345, "R Table"=w346, "S Table"=w347, "error in"=w340, "Table Tag C"=w348, "TDMSファイル in"=w349) -> ("error out"=w339:errorcluster, "TDMSファイル out"=w350:refnum<k34>)  [unwired: 4 in]
    n311 = property on="TDMS temp refnum" class="Ref (strict)"(error in=w339, "Value"=w350) -> (error out=w338:errorcluster)  [unwired: 1 in, 1 out]
    n312 = property on="Table Pass refnum" class="Clust (strict)"(error in=w338) -> (error out=w334:errorcluster, "Value"=w335:T4)  [unwired: 1 in, 1 out]
    n313 = property on="S Table" class="Tbl (strict)"(error in=w334) -> (error out=w333:errorcluster, "Value"=w330:string[][])  [unwired: 1 in, 1 out]
    n314 = property on="B Table" class="Tbl (strict)"(error in=w333) -> (error out=w332:errorcluster, "Value"=w328:string[][])  [unwired: 1 in, 1 out]
    n315 = property on="R Table" class="Tbl (strict)"(error in=w332) -> (error out=w331:errorcluster, "Value"=w329:string[][])  [unwired: 1 in, 1 out]
    n316 = call "anal txt each save.vi"("B Table"=w328, "R Table"=w329, "S Table"=w330, "error in"=w331, "Table Pass refnum_in"=w335) -> ("error out"=w337:errorcluster, "Table Pass refnum_out"=w336:T4)  [unwired: 5 in]
    n317 = property on="Table Pass refnum" class="Clust (strict)"("Value"=w336) -> ()  [unwired: 2 in, 2 out]
    n318 = property on="before" class="Str"(error in=w337) -> (error out=w447:errorcluster, "Value"=w456:string)  [unwired: 1 in, 1 out]
    n319 = Get Date/Time In Seconds() -> (seconds since 1Jan1904=w449:timestamp)
    n320 = call "ANAL Time date.vi"("タイムスタンプ"=w449, "Before"=w456) -> ("Anal Time"=w448:string)  [unwired: 9 in]
    n321 = property on="Anal Time" class="Str"(error in=w447, "Value"=w448) -> (error out=w439:errorcluster)  [unwired: 1 in, 1 out]
    "Rigon#" <- w605
  }
  n322 = property on="Region BL" class="Arr (strict)"(error in=w68) -> (error out=w75:errorcluster, "Value"=w72:dbl[])  [unwired: 1 in, 1 out]
  n323 = property on="Region STD" class="Arr (strict)"(error in=w75) -> (error out=w67:errorcluster, "Value"=w73:dbl[])  [unwired: 1 in, 1 out]
  n324 = property on="Region Count" class="Arr (strict)"(error in=w67) -> (error out=w66:errorcluster, "Value"=w74:dbl[])  [unwired: 1 in, 1 out]
  n325 = call "R Table Graph VI.vi"("R Signal Count"=w74, "Region STD"=w73, "Region BL"=w72) -> ("Count Graph"=→"Count Graph":cluster{i32[], "Count":dbl[]}[], "STDW Graph"=→"STD Graph":cluster{i32[], "Count":dbl[]}[], "BLW Graph"=→"BL Graph":cluster{i32[], "Count":dbl[]}[])  [unwired: 6 in]
  n326 = property on="Anal Time" class="Str"(error in=w66) -> (error out=w151:errorcluster, "Value"=w150:string)  [unwired: 1 in, 1 out]
  n327 = property on="Filename" class="Str"(error in=w151) -> (error out=w158:errorcluster, "Value"=w152:string)  [unwired: 1 in, 1 out]
  n328 = property on="Region STD" class="Arr (strict)"(error in=w158) -> (error out=w159:errorcluster, "Value"=w157:dbl[])  [unwired: 1 in, 1 out]
  n329 = property on="Region Count" class="Arr (strict)"(error in=w159) -> (error out=w160:errorcluster, "Value"=w155:dbl[])  [unwired: 1 in, 1 out]
  n330 = property on="Region BL" class="Arr (strict)"(error in=w160) -> (error out=w161:errorcluster, "Value"=w156:dbl[])  [unwired: 1 in, 1 out]
  n331 = property on="1s datapoint" class="DigNum (strict)"(error in=w161) -> (error out=w148:errorcluster, "Value"=w147:i32)  [unwired: 1 in, 1 out]
  n332 = property on="Rigon#" class="DigNum (strict)"(error in=w148) -> (error out=w149:errorcluster, "Value"=w145:i32)  [unwired: 1 in, 1 out]
  n333 = property on="Read Region Point" class="DigNum (strict)"(error in=w149) -> (error out=w163:errorcluster, "Value"=w146:i32)  [unwired: 1 in, 1 out]
  n334 = property on="B Region Time [s] in" class="DigNum (strict)"(error in=w163) -> (error out=w164:errorcluster, "Value"=w162:dbl)  [unwired: 1 in, 1 out]
  n335 = Bundle("Value"=w150, "Value"=w152) -> (w153:cluster{"Value":string, "Value":string})  [unwired: 1 in]
  n336 = call "ASD total S analysis.vi"("AF_C"=w153, "1s datapoint"=w147, "Read Region Point"=w146, "B Region Time [s] in"=w162, "Rigon#"=w145, "Region Count"=w155, "Region STD"=w157, "Region BL"=w156) -> ("A Cluster"=w154:T16)  [unwired: 3 in]
  n337 = property on="A Cluster" class="Clust (strict)"(error in=w164, "Value"=w154) -> (error out=w98:errorcluster)  [unwired: 1 in, 1 out]
  n338 = Current VI's Path() -> (path=w168:path)
  n339 = property on="info Cluster" class="Clust (strict)"(error in=w98) -> (error out=w97:errorcluster, "Value"=w107:T9)  [unwired: 1 in, 1 out]
  n340 = property on="Burst#Sum" class="DigNum (strict)"(error in=w97) -> (error out=w181:errorcluster, "Value"=w187:i32)  [unwired: 1 in, 1 out]
  n341 = property on="Signal#Sum" class="DigNum (strict)"(error in=w181) -> (error out=w180:errorcluster, "Value"=w186:i32)  [unwired: 1 in, 1 out]
  n342 = property on="R B_SCount [n] in" class="DigNum (strict)"(error in=w180) -> (error out=w179:errorcluster, "Value"=w185:i32)  [unwired: 1 in, 1 out]
  n343 = property on="B Region Time [s] in" class="DigNum (strict)"(error in=w179) -> (error out=w178:errorcluster, "Value"=w184:dbl)  [unwired: 1 in, 1 out]
  n344 = property on="Signal Freq [/s]" class="DigNum (strict)"(error in=w178) -> (error out=w177:errorcluster, "Value"=w183:dbl)  [unwired: 1 in, 1 out]
  n345 = property on="datapoint" class="DigNum (strict)"(error in=w177) -> (error out=w176:errorcluster, "Value"=w182:i32)  [unwired: 1 in, 1 out]
  n346 = property on="A Cluster" class="Clust (strict)"(error in=w176) -> (error out=w104:errorcluster, "Value"=w105:T16)  [unwired: 1 in, 1 out]
  n347 = property on="Selection" class="Enum (strict)"(error in=w104) -> (error out=w103:errorcluster, "Value"=w172:enum16{"10kHz", "100kHz"})  [unwired: 1 in, 1 out]
  n348 = Strip Path(path=w168) -> (name=w171:string)  [unwired: 1 out]
  n349 = call "GetFileCreationDate.vi"("File Path"=w168) -> ("File Created Date (UTC)"=w167:timestamp)  [unwired: 7 in, 1 out]
  n350 = Format Date/Time String(time format string (%c)="%Y_%m%d_%H:%M:%S" ("時間形式文字列（%c）"), seconds (now)=w167) -> (date/time string=w166:string)  [unwired: 1 in]
  n351 = Match Pattern(string=w171, regular expression=".vi" ("正規表現")) -> (before substring=w169:string)  [unwired: 1 in, 3 out]
  n352 = Bundle("Value"=w172, "name"=w169, "date/time string"=w166) -> (w18:T40)  [unwired: 1 in]
  "AA2 info" <- w18
  n353 = Bundle("Value"=w187, "Value"=w186, "Value"=w185, "Value"=w184, "Value"=w183, "Value"=w182) -> (w106:T41)  [unwired: 1 in]
  "AA info" <- w106
  n354 = call "AR table formation VI.vi"("AA2 info"=w18, "A Cluster"=w105, "AA info"=w106, "info Cluster"=w107) -> ("AR Table Data"=w108:string[])  [unwired: 7 in]
  n355 = property on="AR Table Data" class="Arr (strict)"(error in=w103, "Value"=w108) -> (error out=w102:errorcluster)  [unwired: 1 in, 1 out]
  n356 = property on="TDMS temp refnum" class="Ref (strict)"(error in=w102) -> (error out=w101:errorcluster, "Value"=w116:refnum<k34>)  [unwired: 1 in, 1 out]
  n357 = property on="AR Table Tag" class="Arr (strict)"(error in=w101) -> (error out=w100:errorcluster, "Value"=w110:string[])  [unwired: 1 in, 1 out]
  n358 = property on="AR Table Data" class="Arr (strict)"(error in=w100) -> (error out=w99:errorcluster, "Value"=w109:string[])  [unwired: 1 in, 1 out]
  n359 = call "AR Table save for TDMS.vi"("error in"=w99, "AR Table Data"=w109, "AR Table Tag"=w110, "TDMSファイル in"=w116) -> ("error out"=w114:errorcluster, "TDMSファイル out"=w115:refnum<k34>)  [unwired: 6 in]
  n360 = property on="TDMS temp refnum" class="Ref (strict)"(error in=w114, "Value"=w115) -> (error out=w96:errorcluster)  [unwired: 1 in, 1 out]
  n361 = property on="S Table refnum" class="Ref (strict)"(error in=w96) -> (error out=w296:errorcluster, "Value"=w91:refnum<file>)  [unwired: 1 in, 1 out]
  n362 = property on="B Table refnum" class="Ref (strict)"(error in=w296) -> (error out=w295:errorcluster, "Value"=w89:refnum<file>)  [unwired: 1 in, 1 out]
  n363 = property on="R Table refnum" class="Ref (strict)"(error in=w295) -> (error out=w95:errorcluster, "Value"=w90:refnum<file>)  [unwired: 1 in, 1 out]
  n364 = property on="TDMS temp refnum" class="Ref (strict)"(error in=w95) -> (error out=w94:errorcluster, "Value"=w92:refnum<k34>)  [unwired: 1 in, 1 out]
  n365 = call "Anal tzt close header_MS.vi"("A TDMS refnum"=w92, "error in"=w94, "B Table refnum"=w89, "R Table refnum"=w90, "S Table refnum"=w91) -> ("error out"=w93:errorcluster)  [unwired: 6 in]
  n366 = Current VI's Path() -> (path=w288:path)
  n367 = property on="JPEG Path" class="Path"(error in=w93) -> (error out=w293:errorcluster, "Value"=w292:path)  [unwired: 1 in, 1 out]
  n368 = call "Front Panel JPEG file converter.vi"("error in"=w293, "JPEG file name"=w292, "VI Path"=w288) -> ("error out"=w53:errorcluster)  [unwired: 8 in]
  n369 = property on="tdms tmp path" class="Path"(error in=w53) -> (error out=w51:errorcluster, "Value"=w38:path)  [unwired: 1 in, 1 out]
  n370 = property on="A TDMS Path" class="Path"(error in=w51) -> (error out=w52:errorcluster, "Value"=w39:path)  [unwired: 1 in, 1 out]
  n371 = Copy(8:w52, 10:w39, 11:w38) -> (0:w5:errorcluster)  [unwired: 2 in, 2 out]
  n372 = Strip Path(path=w38) -> (stripped path=w9:path)  [unwired: 1 out]
  n373 = call <vilib>:"Clear Errors.vi"("error in (no error)"=w5, "specific error code to clear (0: all)"=6) -> ("error out"=w4:errorcluster)  [unwired: 4 in, 1 out]
  n374 = property on="stripped path" class="Path"(error in=w4, "Value"=w9) -> (error out=w10:errorcluster)  [unwired: 1 in, 1 out]
  n375 = property on="A New Folder temp" class="Str"(error in=w10) -> (error out=w34:errorcluster, "Value"=w24:string)  [unwired: 1 in, 1 out]
  n376 = property on="A New folder" class="Str"(error in=w34) -> (error out=w33:errorcluster, "Value"=w23:string)  [unwired: 1 in, 1 out]
  n377 = Reverse String(1:w23) -> (0:w31:string)
  n378 = Reverse String(1:w24) -> (0:w27:string)
  n379 = Match Pattern(string=w31, regular expression="\\") -> (after substring=w30:string)  [unwired: 1 in, 3 out]
  n380 = Match Pattern(string=w27, regular expression="\\") -> (after substring=w26:string)  [unwired: 1 in, 3 out]
  n381 = Reverse String(1:w30) -> (0:w29:string)
  n382 = Reverse String(1:w26) -> (0:w25:string)
  n383 = String To Path(string=w29) -> (path=w21:path)
  n384 = Strip Path(path=w21) -> (stripped path=w19:path)  [unwired: 1 out]
  "path 2" <- w19
  n385 = String To Path(string=w25) -> (path=w22:path)
  "path" <- w22
  n386 = Copy(8:w33, 9:TRUE ("overwrite (F)"), 10:w19, 11:w22) -> (0:w11:errorcluster)  [unwired: 1 in, 2 out]
  n387 = while {
    tunnel: w11 -> [w671]
    tunnel: [w671] -> w7
    i -> [w670]
    stop <- w668 stop-if-true
    n388 = Equal?(x=w670, y=2) -> (x = y?=w668:bool)
    n389 = Wait (ms)(milliseconds to wait=u32 1000 ("millisecond timer value")) -> ()  [unwired: 1 out]
  }
  n390 = property on="stripped path" class="Path"(error in=w7) -> (error out=w6:errorcluster, "Value"=w8:path)  [unwired: 1 in, 1 out]
  n391 = Delete(path (use dialog)=w8, entire hierarchy (F)=TRUE, error in=w6) -> (error out=→"error out":errorcluster)  [unwired: 2 in, 2 out]
